vi "PhotonTrackedTarget_CreateFromPacket.vi"(9 "StartByte":i32, 11 "RawData":u8[](array[numeric])) -> (1 "NextByte":i32, 3 "TrackedTarget":T1={"Yaw"=0.0, "Pitch"=0.0, "Area"=0.0, "Skew"=0.0, "TargetCorners"=[], "CameraToTarget"={"TRANSLATION"={"X"=0.0, "Y"=0.0}, "ROTATION"={"VALUE"=0.0, "COS"=1.0, "SIN"=0.0}}} {"CameraToTarget"."ROTATION"."SIN" format="%13.4f"; "CameraToTarget"."ROTATION"."COS" format="%13.4f"; "CameraToTarget"."ROTATION"."VALUE" format="%13.4f"; "CameraToTarget"."TRANSLATION"."Y" format="%14.3f"; "CameraToTarget"."TRANSLATION"."X" format="%14.3f"})   [LabVIEW 2019, in "PhotonVisionLib.lvlib"]
doc: "Internal function to parse the data for each target returned by PhotonCamera_GetLatestResult.\n\nInputs:\n - RawData -- Byte array containing the data to parse.\n\nOutputs:\n - TrackedTarget -- Parsed TrackedTarget cluster."
uses:
  PhotonVisionLib.lvlib
  TypeDef/PhotonTrackedTargetType.ctl
  TypeDef/TargetCornerType.ctl
  <vilib>/Rock Robotics/WPI/ThirdParty/JAS_Junk/TrajLib/TRANSFORM2D.ctl
  <vilib>/Rock Robotics/WPI/ThirdParty/JAS_Junk/TrajLib/TRANSLATION2D.ctl
  <vilib>/Rock Robotics/WPI/ThirdParty/JAS_Junk/TrajLib/ROTATION2D.ctl
  <vilib>/Rock Robotics/WPI/ThirdParty/JAS_Junk/TrajLib/Conv_Deg_Radians.vi
  <vilib>/Rock Robotics/WPI/ThirdParty/JAS_Junk/TrajLib/Rotation2d_CreateAngle.vi
  <vilib>/Rock Robotics/WPI/ThirdParty/JAS_Junk/TrajLib/Trajectory_Library.lvlib
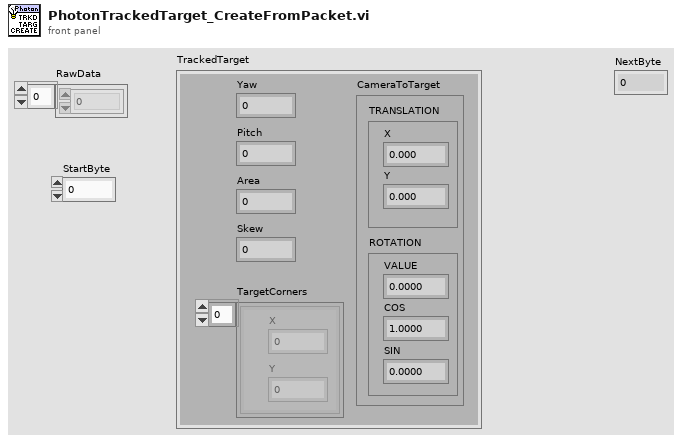
[diagram p1: front panel]
types:
  T1 = typedef "PhotonVisionLib.lvlib/PhotonTrackedTargetType.ctl" = cluster{"Yaw":dbl, "Pitch":dbl, "Area":dbl, "Skew":dbl, "TargetCorners":T2[], "CameraToTarget":T3}
  T2 = typedef "PhotonVisionLib.lvlib/TargetCornerType.ctl" = cluster{"X":dbl, "Y":dbl}
  T3 = typedef "Trajectory_Library.lvlib/TRANSFORM2D.ctl" = cluster{"TRANSLATION":T4, "ROTATION":T5}
  T4 = typedef "Trajectory_Library.lvlib/TRANSLATION2D.ctl" = cluster{"X":dbl, "Y":dbl}
  T5 = typedef "Trajectory_Library.lvlib/ROTATION2D.ctl" = cluster{"VALUE":dbl, "COS":dbl, "SIN":dbl}
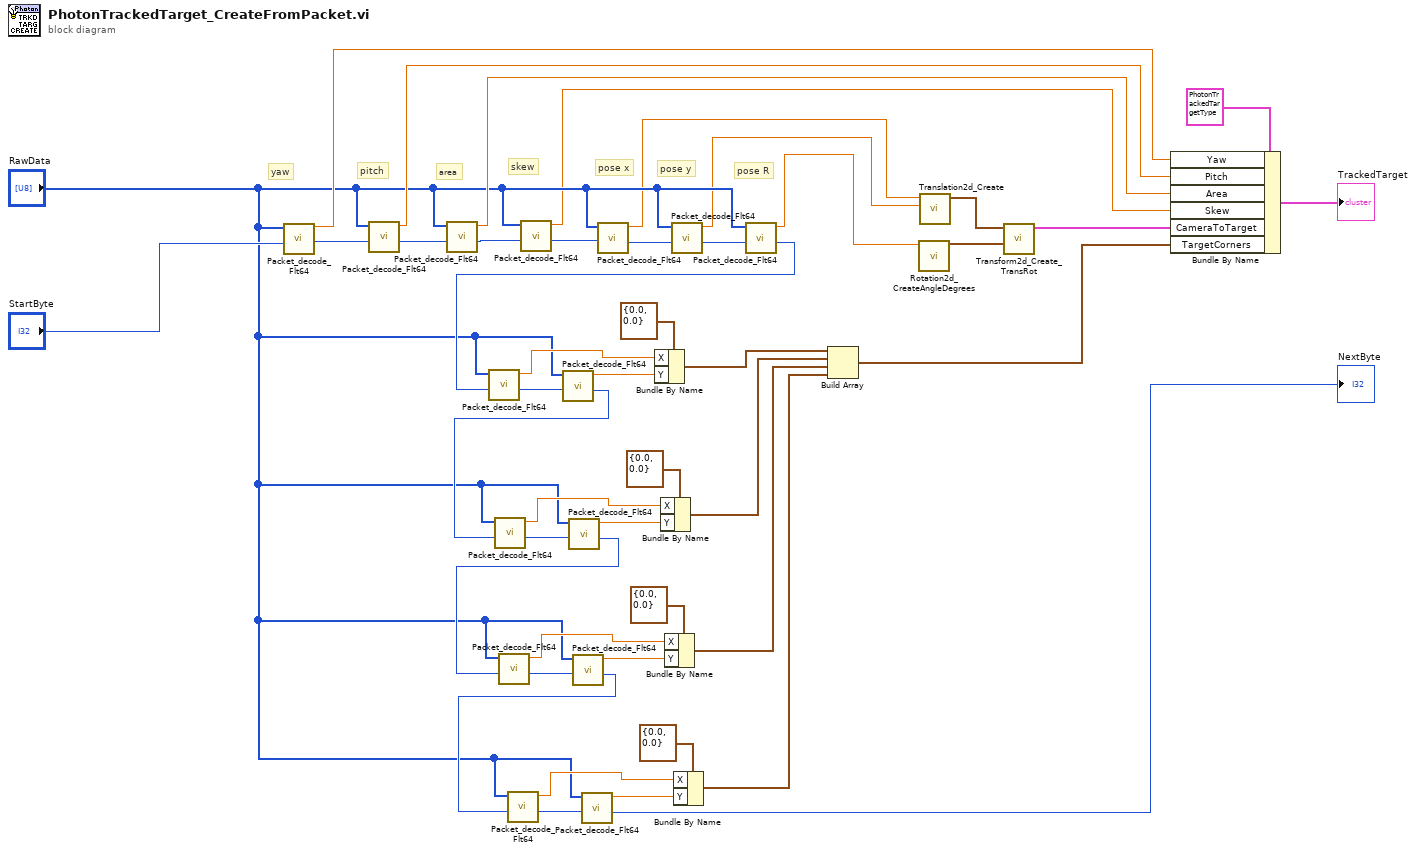
[diagram p0: block diagram]
diagram:
  # "pose R"
  # "pose y"
  # "pose x"
  # "skew"
  # "area"
  # "pitch"
  # "yaw"
  n1 = call "Packet_decode_Flt64.vi"("StartByte"="StartByte", "RawData"="RawData") -> ("NextByte"=w43:i32, "Flt64_Value"=w46:dbl)  [unwired: 8 in]
  n2 = call "Packet_decode_Flt64.vi"("StartByte"=w43, "RawData"="RawData") -> ("NextByte"=w41:i32, "Flt64_Value"=w42:dbl)  [unwired: 8 in]
  n3 = call "Packet_decode_Flt64.vi"("StartByte"=w41, "RawData"="RawData") -> ("NextByte"=w10:i32, "Flt64_Value"=w17:dbl)  [unwired: 8 in]
  n4 = call "Packet_decode_Flt64.vi"("StartByte"=w10, "RawData"="RawData") -> ("NextByte"=w9:i32, "Flt64_Value"=w7:dbl)  [unwired: 8 in]
  n5 = call "Packet_decode_Flt64.vi"("StartByte"=w9, "RawData"="RawData") -> ("NextByte"=w40:i32, "Flt64_Value"=w5:dbl)  [unwired: 8 in]
  n6 = call "Packet_decode_Flt64.vi"("StartByte"=w40, "RawData"="RawData") -> ("NextByte"=w39:i32, "Flt64_Value"=w4:dbl)  [unwired: 8 in]
  n7 = call "Packet_decode_Flt64.vi"("StartByte"=w39, "RawData"="RawData") -> ("NextByte"=w16:i32, "Flt64_Value"=w3:dbl)  [unwired: 8 in]
  n8 = call "Packet_decode_Flt64.vi"("StartByte"=w16, "RawData"="RawData") -> ("NextByte"=w38:i32, "Flt64_Value"=w35:dbl)  [unwired: 8 in]
  n9 = call "Packet_decode_Flt64.vi"("StartByte"=w38, "RawData"="RawData") -> ("NextByte"=w15:i32, "Flt64_Value"=w36:dbl)  [unwired: 8 in]
  n10 = call "Packet_decode_Flt64.vi"("StartByte"=w15, "RawData"="RawData") -> ("NextByte"=w34:i32, "Flt64_Value"=w31:dbl)  [unwired: 8 in]
  n11 = call "Packet_decode_Flt64.vi"("StartByte"=w34, "RawData"="RawData") -> ("NextByte"=w14:i32, "Flt64_Value"=w32:dbl)  [unwired: 8 in]
  n12 = call "Packet_decode_Flt64.vi"("StartByte"=w14, "RawData"="RawData") -> ("NextByte"=w30:i32, "Flt64_Value"=w27:dbl)  [unwired: 8 in]
  n13 = call "Packet_decode_Flt64.vi"("StartByte"=w30, "RawData"="RawData") -> ("NextByte"=w13:i32, "Flt64_Value"=w28:dbl)  [unwired: 8 in]
  n14 = call "Packet_decode_Flt64.vi"("StartByte"=w13, "RawData"="RawData") -> ("NextByte"=w26:i32, "Flt64_Value"=w23:dbl)  [unwired: 8 in]
  n15 = call "Packet_decode_Flt64.vi"("StartByte"=w26, "RawData"="RawData") -> ("NextByte"=→"NextByte":i32, "Flt64_Value"=w24:dbl)  [unwired: 8 in]
  n16 = Bundle By Name(cluster=T2 {"X"=0.0, "Y"=0.0} ("TargetCorner"), "X"=w35, "Y"=w36) -> (w22:T2)
  n17 = Bundle By Name(cluster=T2 {"X"=0.0, "Y"=0.0} ("TargetCorner"), "X"=w31, "Y"=w32) -> (w21:T2)
  n18 = Bundle By Name(cluster=T2 {"X"=0.0, "Y"=0.0} ("TargetCorner"), "X"=w27, "Y"=w28) -> (w20:T2)
  n19 = Bundle By Name(cluster=T2 {"X"=0.0, "Y"=0.0} ("TargetCorner"), "X"=w23, "Y"=w24) -> (w19:T2)
  n20 = Build Array(w22, w21, w20, w19) -> (w18:T2[])
  n21 = call <vilib>:"Rotation2d_CreateAngleDegrees.vi"("Angle_Degrees"=w3) -> ("ROTATION"=w2:T5)  [unwired: 10 in]
  n22 = call <vilib>:"Translation2d_Create.vi"("Y"=w4, "X"=w5) -> ("TRANSLATION"=w1:T4)  [unwired: 9 in]
  n23 = call <vilib>:"Transform2d_Create_TransRot.vi"("ROTATION"=w2, "TRANSLATION"=w1) -> ("TRANSFORM"=w6:T3)  [unwired: 9 in]
  n24 = Bundle By Name(cluster=T1 {"Yaw"=0.0, "Pitch"=0.0, "Area"=0.0, "Skew"=0.0, "TargetCorners"=[], "CameraToTarget"={"TRANSLATION"={"X"=0.0, "Y"=0.0}, "ROTATION"={"VALUE"=0.0, "COS"=1.0, "SIN"=0.0}}} ("PhotonTrackedTarget"), "Yaw"=w46, "Pitch"=w42, "Area"=w17, "Skew"=w7, "CameraToTarget"=w6, "TargetCorners"=w18) -> (→"TrackedTarget":T1)
